vi "Lab4_task5 (1).vi"() -> ()   [LabVIEW 2022 SP3]
uses:
  <vilib>/Analysis/baseanly.llb/Mean (DBL).vi
  <vilib>/Analysis/5stat.llb/RMS (DBL).vi
  <vilib>/Utility/file.llb/Write Delimited Spreadsheet (DBL).vi
  <vilib>/express/express analysis/Spectral/Block/exnSpectralBlock spectral measurements PSD poly.vi
  <vilib>/express/express analysis/Spectral/Block/exnSpectralBlock spectral measurements PSD DDT.vi
  <vilib>/express/express analysis/Spectral/XNode/ExpressSpectralMeasurementsBlockNode.xnode
  <vilib>/Analysis/NI_AALBase.lvlib
  <vilib>/Analysis/NI_AALPro.lvlib
panel:
  in  "file path (dialog if empty)":path
  in  "stop 2":bool
  out "Array":dbl[](array[numeric])
  out "Intensity Chart":dbl[][](graph)
  in  "stop":bool
  in  "number of samples":i32=100000
  out "PSD":dynamicdata(graph)
  in  "Sampling rate (Hz)":dbl
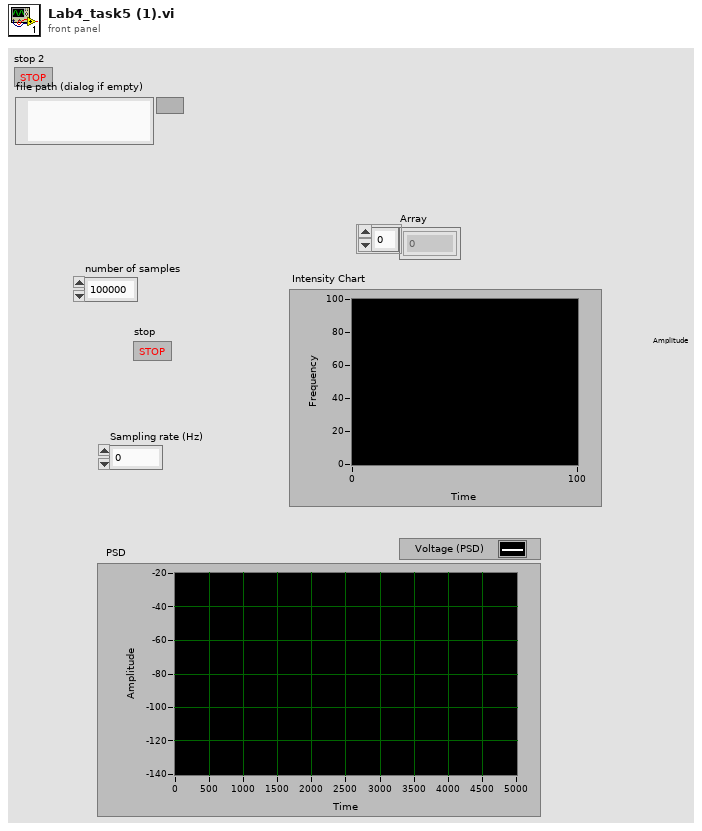
[diagram p1: front panel]
types:
  T1 = cluster{"averaging mode":u16, "weighting mode":u16, "number of averages":u32}
  T2 = cluster{"dB On (F)":bool, "unwrap phase (F)":bool, "convert to degree (F)":bool}
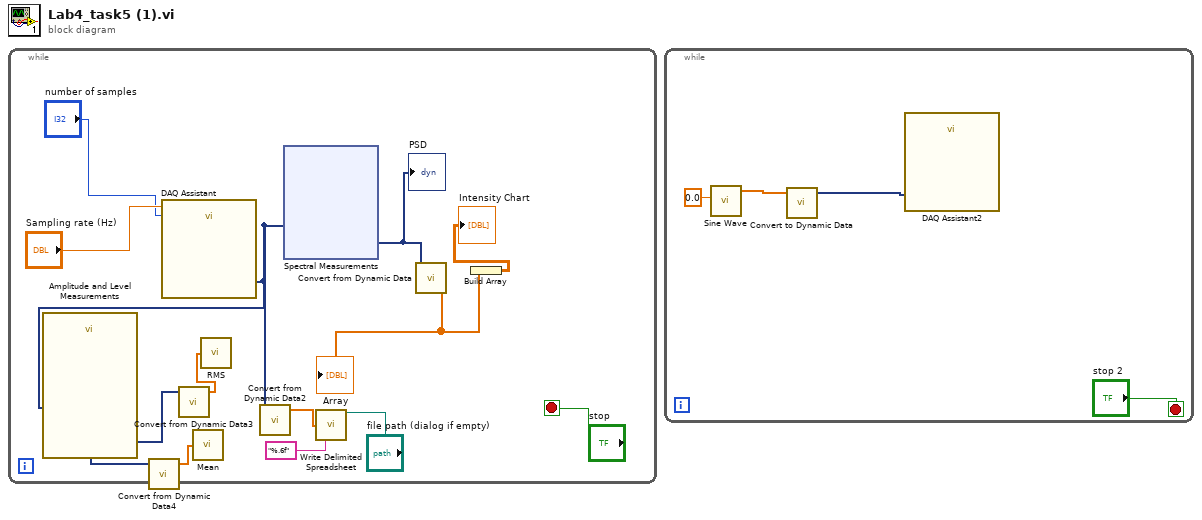
[diagram p0: block diagram]
diagram:
  n1 = while {
    stop <- "stop" stop-if-true
    n2 = call "DAQ Assistant"("rate"="Sampling rate (Hz)", "number of samples"="number of samples") -> ("data"=w9:dynamicdata)  [unwired: 15 in, 2 out]
    n3 = call "Amplitude and Level Measurements"("Signals"=w9) -> ("RMS"=w5:dynamicdata, "Peak to Peak"=w3:dynamicdata)  [unwired: 12 in, 1 out]
    n4 = call "Convert from Dynamic Data4"("Dynamic Data Type"=w3) -> ("Array"=w2:dbl[])  [unwired: 3 in]
    n5 = call "Convert from Dynamic Data3"("Dynamic Data Type"=w5) -> ("Array"=w4:dbl[])  [unwired: 3 in]
    n6 = call-poly <vilib>:"Mean.vi"("X"=w2) -> ()  [unwired: 2 out]
    n7 = call-poly <vilib>:"RMS.vi"("X"=w4) -> ()  [unwired: 2 out]
    n8 = call "Convert from Dynamic Data2"("Dynamic Data Type"=w9) -> ("Array"=w6:dbl[])  [unwired: 3 in]
    n9 = xnode "Spectral Measurements"("Signals"=w9) -> ("PSD"=w12:dynamicdata)  [unwired: 1 in, 1 out]
    "PSD" <- w12
    n10 = call-poly <vilib>:"Write Delimited Spreadsheet.vi"("file path (dialog if empty)"="file path (dialog if empty)", "format (%.6f)"="%.6f", "1D data"=w6) -> ()  [unwired: 11 in, 2 out]
    n11 = call "Convert from Dynamic Data"("Dynamic Data Type"=w12) -> ("Array"=w11:dbl[])  [unwired: 3 in]
    "Array" <- w11
    n12 = Build Array(w11) -> (→"Intensity Chart":dbl[][])
  }
  n13 = while {
    stop <- "stop 2" stop-if-true
    n14 = call <vilib>:"Sine Wave.vi"("amplitude"=0.0) -> ("sine wave"=w27:dbl[])  [unwired: 4 in, 2 out]
    n15 = call "Convert to Dynamic Data"("Array"=w27) -> ("Dynamic Data Type"=w26:dynamicdata)  [unwired: 3 in]
    n16 = call "DAQ Assistant2"("data"=w26) -> ()  [unwired: 16 in, 3 out]
  }
